vi "Progress_show.vi"(8 "P_folder names":string[](array[string]), 11 "folder names":string[](array[string])) -> (0 "Array":bool[](array[boolean]), 1 "overlapped array":string[](array[string]), 2 "non-overlapped array":string[](array[string]), 3 "Array 3":cluster{string, bool}[](array[cluster]))   [LabVIEW 2018]
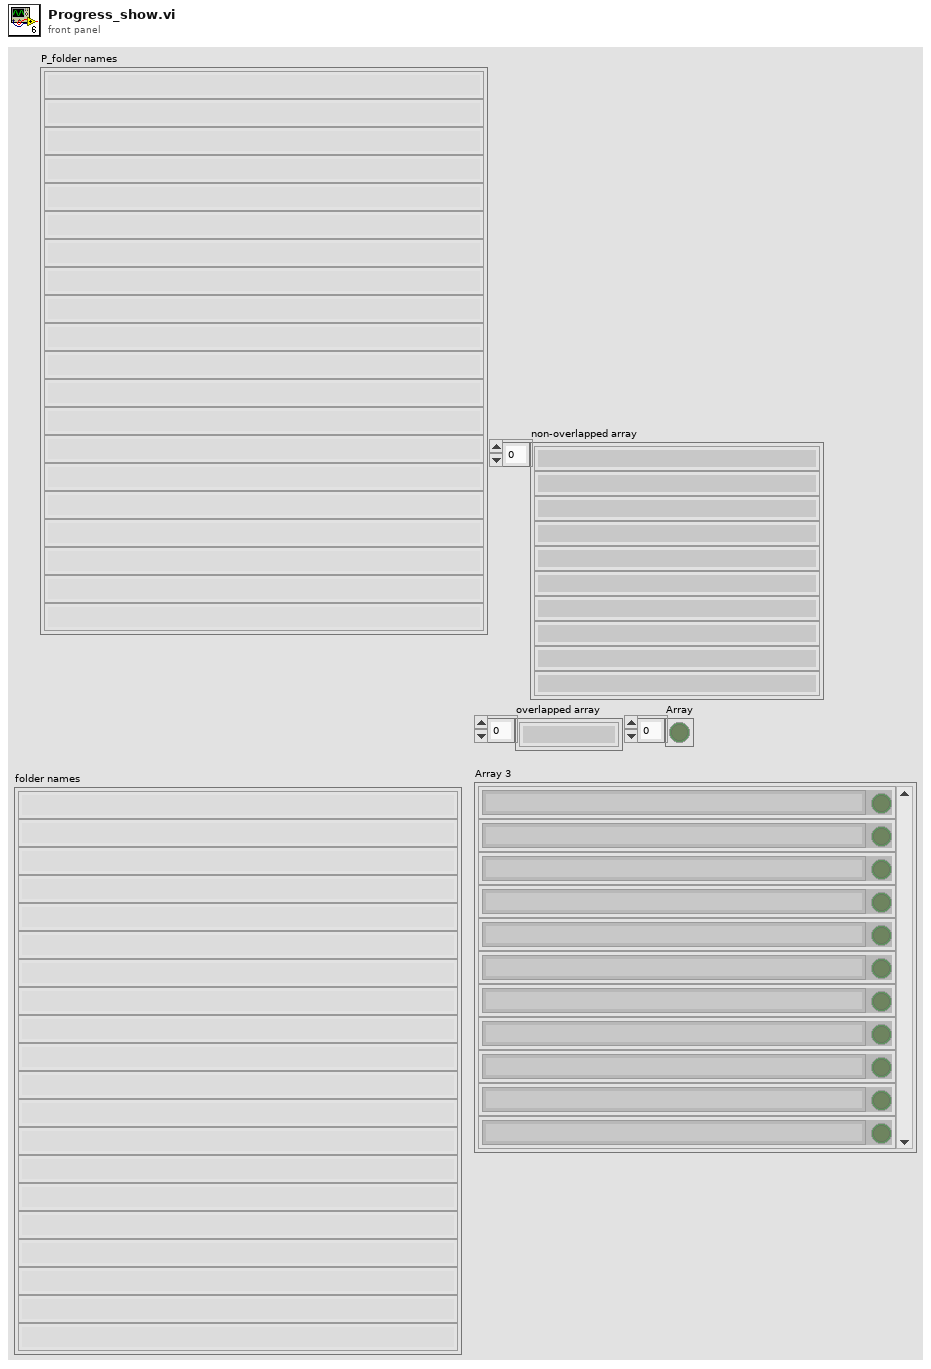
[diagram p1: front panel]
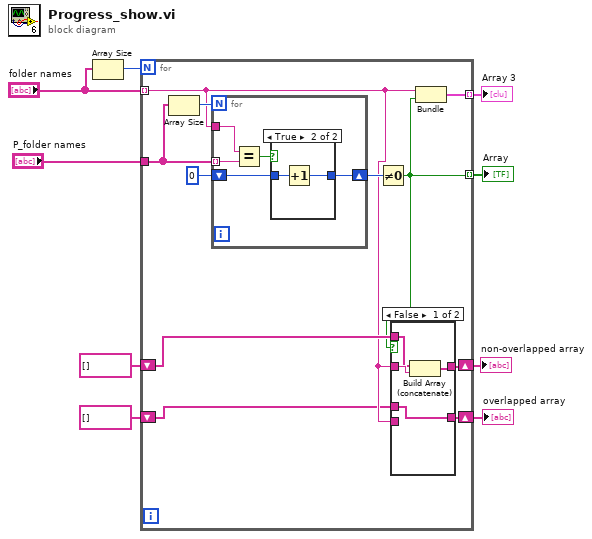
[diagram p0: block diagram]
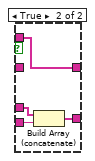
[diagram p2: hidden frame]
diagram:
  n1 = Array Size(array="folder names") -> (size(s)=w9:i32)
  n2 = for {
    N: w9 -> [_]
    tunnel: "P_folder names" -> [w19]
    tunnel: "folder names" -> [w13] mode=indexing
    tunnel: [w16] -> w8 mode=indexing
    shift-right: [w15] -> w4
    shift-left: string[] [] -> [w14]
    shift-right: [w12] -> w2
    shift-left: string[] [] -> [w11]
    tunnel: [w10] -> w1 mode=indexing
    n3 = Array Size(array=w19) -> (size(s)=w20:i32)
    n4 = for {
      N: w20 -> [_]
      tunnel: w13 -> [w33]
      tunnel: w19 -> [w32] mode=indexing
      shift-right: [w30] -> w17
      shift-left: 0 -> [w29]
      n5 = Equal?(x=w33, y=w32) -> (x = y?=w31:bool)
      n6 = case shown="True" w31 {
        tunnel: [w34 w36] -> w30
        tunnel: w29 -> [w34 w35]
        frame False {
        }
        frame True {
          n7 = Increment(x=w35) -> (x+1=w36:i32)
        }
      }
    }
    n8 = Not Equal To 0?(x=w17) -> (x != 0?=w10:bool)
    n9 = case shown="False" w10 {
      tunnel: [w23 w28] -> w15
      tunnel: w13 -> [w24 _]
      tunnel: w14 -> [w22 w28]
      tunnel: w13 -> [_ w27]
      tunnel: [w21 w26] -> w12
      tunnel: w11 -> [w21 w25]
      frame False {
        n10 = Build Array (concatenate)(w22, w24) -> (w23:string[])
      }
      frame True {
        n11 = Build Array (concatenate)(w25, w27) -> (w26:string[])
      }
    }
    n12 = Bundle(w13, w10) -> (w16:cluster{string, bool})  [unwired: 1 in]
  }
  "Array 3" <- w8
  "non-overlapped array" <- w4
  "overlapped array" <- w2
  "Array" <- w1
